vi "list_items.vi"(8 "error in (no error)":errorcluster, 11 "Table in":refnum<class "InlineTable.lvclass">) -> (0 "error out":errorcluster, 2 "items":string[](array[string]), 3 "Table out":refnum<class "InlineTable.lvclass">)   [LabVIEW 2020, in "toml_edit.lvlib" / "InlineTable.lvclass"]
uses:
  InlineTable.lvclass
  InlineTable.lvclass/InlineTable.ctl
  toml_edit.lvlib
  dragon_toml_64.dll
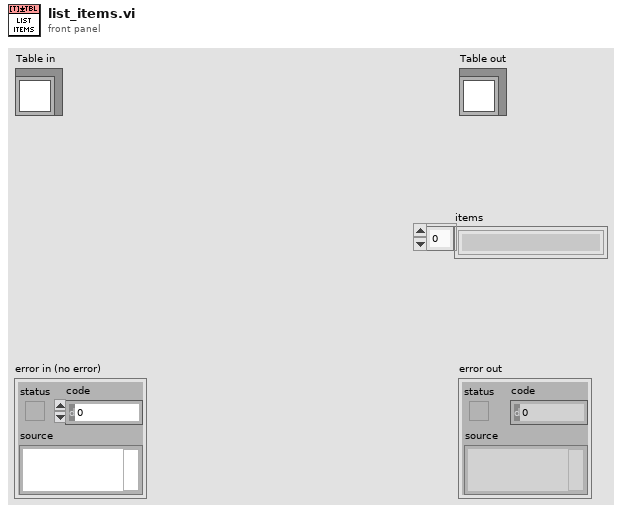
[diagram p1: front panel]
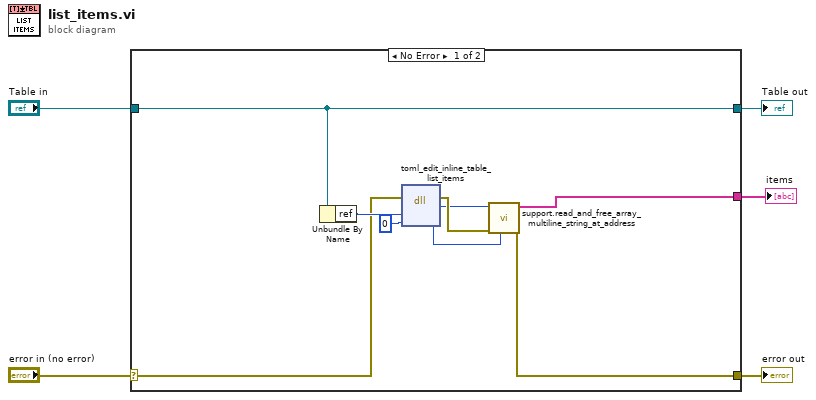
[diagram p0: block diagram]
diagram:
  n1 = case shown="No Error" "error in (no error)" {
    selector: "error in (no error)" -> [w10 w16]
    tunnel: [w9 w16] -> w4
    tunnel: [w11 w15] -> w2
    tunnel: "Table in" -> [w11 w15]
    tunnel: [w8 _] -> w1
    frame No Error {
      n2 = Unbundle By Name(w11) -> ("ref"=w12:u64)
      n3 = dll-call lib="C:/projects/dragon-desktop/source/submodules/toml-edit-labview/lv_src/dragon_toml_*.dll" fn="toml_edit_inline_table_list_items"(error in=w10, "table_ref"=w12, "string_length"=u32 0) -> (error out=w14:errorcluster, "item_names_ptr"=w13:u64, "string_length"=w7:u32)  [unwired: 3 in, 1 out]
      n4 = call "support.read_and_free_array_multiline_string_at_address.vi"("string length"=w7, "error in (no error)"=w14, "table_names_ptr"=w13) -> ("error out"=w9:errorcluster, "lines"=w8:string[])  [unwired: 7 in]
    }
    frame Error {
    }
  }
  "error out" <- w4
  "Table out" <- w2
  "items" <- w1
